vi "Cleanup Session.vi"(8 "error in":errorcluster, 11 "Plugin in":refnum<class "DFT_Spectra.lvclass">) -> (0 "error out":errorcluster, 3 "Plugin out":refnum<class "DFT_Spectra.lvclass">)   [LabVIEW 2024, in "DFT_Spectra.lvlib" / "DFT_Spectra.lvclass"]
uses:
  DFT_Spectra.lvclass
  DFT_Spectra.lvclass/DFT_Spectra.ctl
  <vilib>/addons/_NISVFA/_Shared subVIs/Data Objects/Waveforms (DBL)/Waveforms (N Ch).lvclass
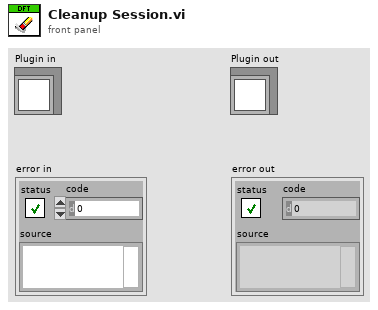
[diagram p1: front panel]
types:
  T1 = enum32{"Invalid", "Standard", "Closed", "Hidden", "Minimized", "Maximized"}
  T2 = typedef "DFT_Spectra.lvlib/DFT_Spectra.lvclass/DFT_Spectra Data.ctl" = cluster{"First Time":bool, "Show Results Window":bool, "Show Results Window Clicked":bool, "Window":T3, "overlap":i32, "Block Duration":dbl, "Averaging parameters":cluster{"averaging mode":enum16{"No averaging", "Vector averaging", "RMS averaging", "Peak hold"}, "weighting mode":enum16{"Linear", "Exponential"}, "number of averages":u32}, "buffer out":refnum<data-value>, "Avg Spectra":refnum<vi>, "Spectra UI":refnum<vi>}
  T3 = typedef "NI_AALPro.lvlib/windowTd.ctl" = u32
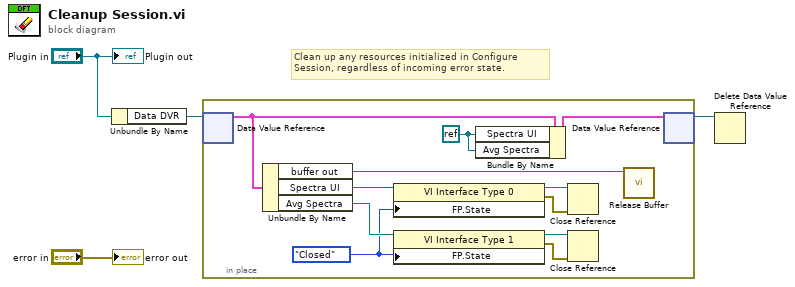
[diagram p0: block diagram]
diagram:
  # "Clean up any resources initialized in Configure Session, regardless of incoming error state."
  n1 = Unbundle By Name("Plugin in") -> ("Data DVR"=w4:refnum<data-value>)
  n2 = in-place {
    w6 = T1."Closed" ("Front Panel Window:State")
    w5 = refnum<k0> refnum
    n3 = in-place-dvr #1(w4) -> (w15:T2)  [unwired: 1 out]
    n4 = Unbundle By Name(w15) -> ("buffer out"=w10:refnum<data-value>, "Spectra UI"=w14:refnum<vi>, "Avg Spectra"=w7:refnum<vi>)
    n5 = property class="VI Interface Type 0"(reference=w14, "FP.State"=w6) -> (reference out=w13:refnum<vi>, error out=w12:errorcluster)  [unwired: 1 in]
    n6 = property class="VI Interface Type 1"(reference=w7, "FP.State"=w6) -> (reference out=w8:refnum<vi>, error out=w9:errorcluster)  [unwired: 1 in]
    n7 = Bundle By Name(cluster=w15, "Spectra UI"=w5, "Avg Spectra"=w5) -> (w11:T2)
    n8 = Close Reference(reference=w13, error in (no error)=w12) -> ()  [unwired: 1 out]
    n9 = Close Reference(reference=w8, error in (no error)=w9) -> ()  [unwired: 1 out]
    n10 = call <vilib>:"Release Buffer.vi"("buffer"=w10) -> ()  [unwired: 10 in, 1 out]
    n11 = in-place-dvr #1(w11) -> (w3:refnum<data-value>)  [unwired: 1 out]
  }
  n12 = Delete Data Value Reference(data value reference=w3) -> ()  [unwired: 1 in, 2 out]
  "error out" <- "error in"
  "Plugin out" <- "Plugin in"
